vi "Find and Rename VIs.vi"(0 "Owned Items[]":refnum<vi>[](array[refnum]), 5 "new name":string, 7 "name to replace":string, 11 "error in":errorcluster) -> (15 "error out":errorcluster)   [LabVIEW 2022 SP3, in "Springboard TLB`.lvlib"]
uses:
  Springboard TLB`.lvlib
  <vilib>/regexp/Match Regular Expression.xnode
panel:
  out "Array 2":string[](array[string])
  out "Array":string[](array[string])
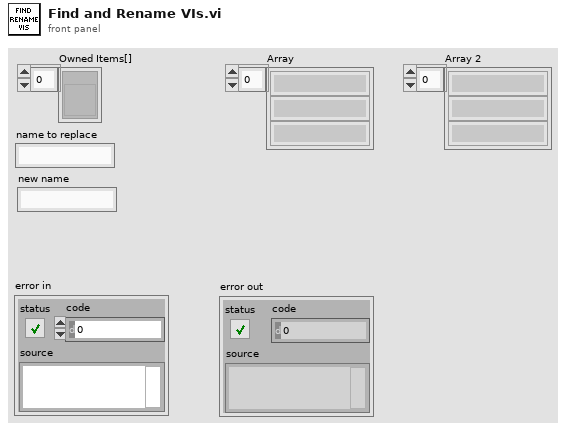
[diagram p1: front panel]
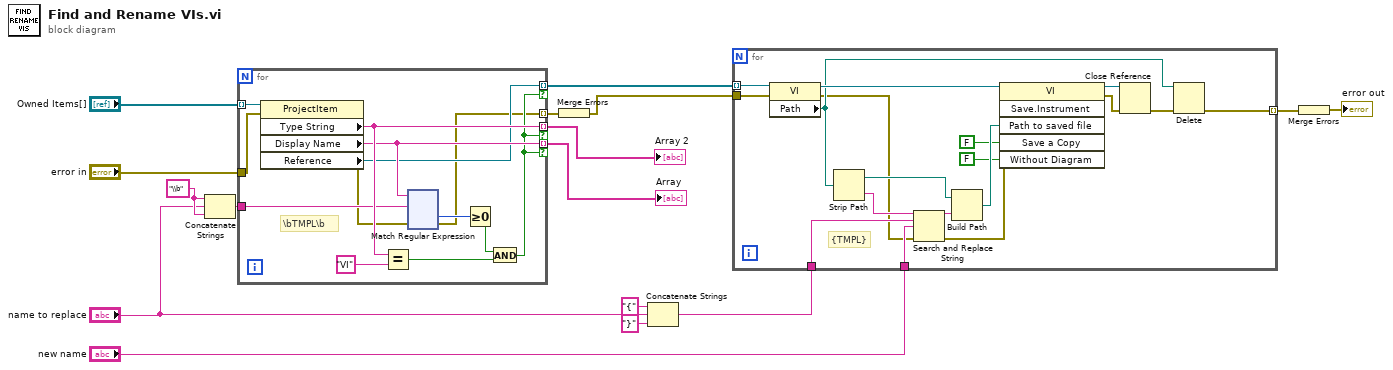
[diagram p0: block diagram]
diagram:
  w5 = "\\b" ("string")
  n1 = Concatenate Strings(w5, "name to replace", w5) -> (w6:string)
  n2 = for {
    tunnel: "Owned Items[]" -> [w29] mode=indexing
    tunnel: [w28] -> w10 mode=indexing if=w22
    tunnel: [w25] -> w11 mode=indexing if=w22
    tunnel: [w21] -> w14 mode=indexing if=w22
    tunnel: [w17] -> w15 mode=indexing
    tunnel: "error in" -> [w20]
    tunnel: w6 -> [w19]
    # "\\bTMPL\\b"
    n3 = property class="ProjectItem"(reference=w29, error in=w20) -> (error out=w18:errorcluster, "Type String"=w28:string, "Display Name"=w25:string, "Reference"=w21:refnum<vi>)  [unwired: 1 out]
    n4 = Equal?(x=w28, y="VI") -> (x = y?=w26:bool)
    n5 = xnode "Match Regular Expression"("input string"=w25, "regular expression"=w19, "error in"=w18) -> ("offset past match"=w24:i32, "error out"=w17:errorcluster)  [unwired: 3 in, 3 out]
    n6 = Greater Or Equal To 0?(x=w24) -> (x >= 0?=w23:bool)
    n7 = And(x=w23, y=w26) -> (x .and. y?=w22:bool)
  }
  "Array" <- w11
  "Array 2" <- w10
  n8 = Merge Errors(w15) -> (w16:errorcluster)
  n9 = Concatenate Strings("{" ("string"), "name to replace", "}" ("string")) -> (w1:string)
  n10 = for {
    tunnel: "new name" -> [w162]
    tunnel: w14 -> [w159] mode=indexing
    tunnel: w16 -> [w154]
    tunnel: [w151] -> w8 mode=indexing
    tunnel: w1 -> [w149]
    # "{TMPL}"
    n11 = property class="VI"(reference=w159, error in=w154) -> (reference out=w164:refnum<vi>, error out=w148:errorcluster, "Path"=w150:path)
    n12 = Strip Path(path=w150) -> (stripped path=w152:path, name=w163:string)
    n13 = Search and Replace String(input string=w163, search string=w149, replace string=w162, error in=w148) -> (result string=w161:string, error out=w147:errorcluster)  [unwired: 4 in, 2 out]
    n14 = Build Path(base path=w152, name or relative path=w161) -> (appended path=w160:path)
    n15 = invoke class="VI" method="Save.Instrument"(reference=w164, error in=w147, "Path to saved file"=w160, "Save a Copy"=FALSE, "Without Diagram"=FALSE) -> (reference out=w156:refnum<vi>, error out=w155:errorcluster)  [unwired: 1 in, 4 out]
    n16 = Close Reference(reference=w156, error in (no error)=w155) -> (error out=w153:errorcluster)
    n17 = Delete(path (use dialog)=w150, error in=w153) -> (error out=w151:errorcluster)  [unwired: 3 in, 2 out]
  }
  n18 = Merge Errors(w8) -> (→"error out":errorcluster)
